vi "Param_Cmds.vi"(4 "Timeout":u16, 5 "Target":u16, 8 "Release":u16, 9 "Vacuum":u16, 10 "Write":bool, 11 "Queue":refnum<queue>) -> ()   [LabVIEW 2026]
doc: "Use this template to build a VI to use as a subVI."
panel:
  # "ÕfÃ÷£º°´ Write r°ÑËÄ¢µÏÞÖÆ¹ úáá·ÅßMÐÁÐ¡£"
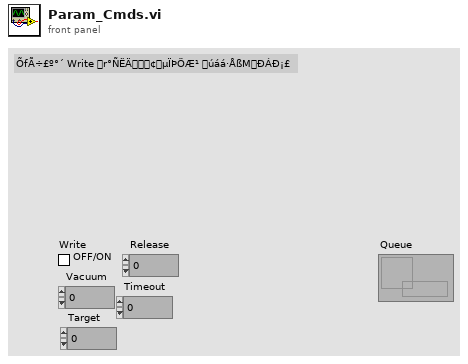
[diagram p1: front panel]
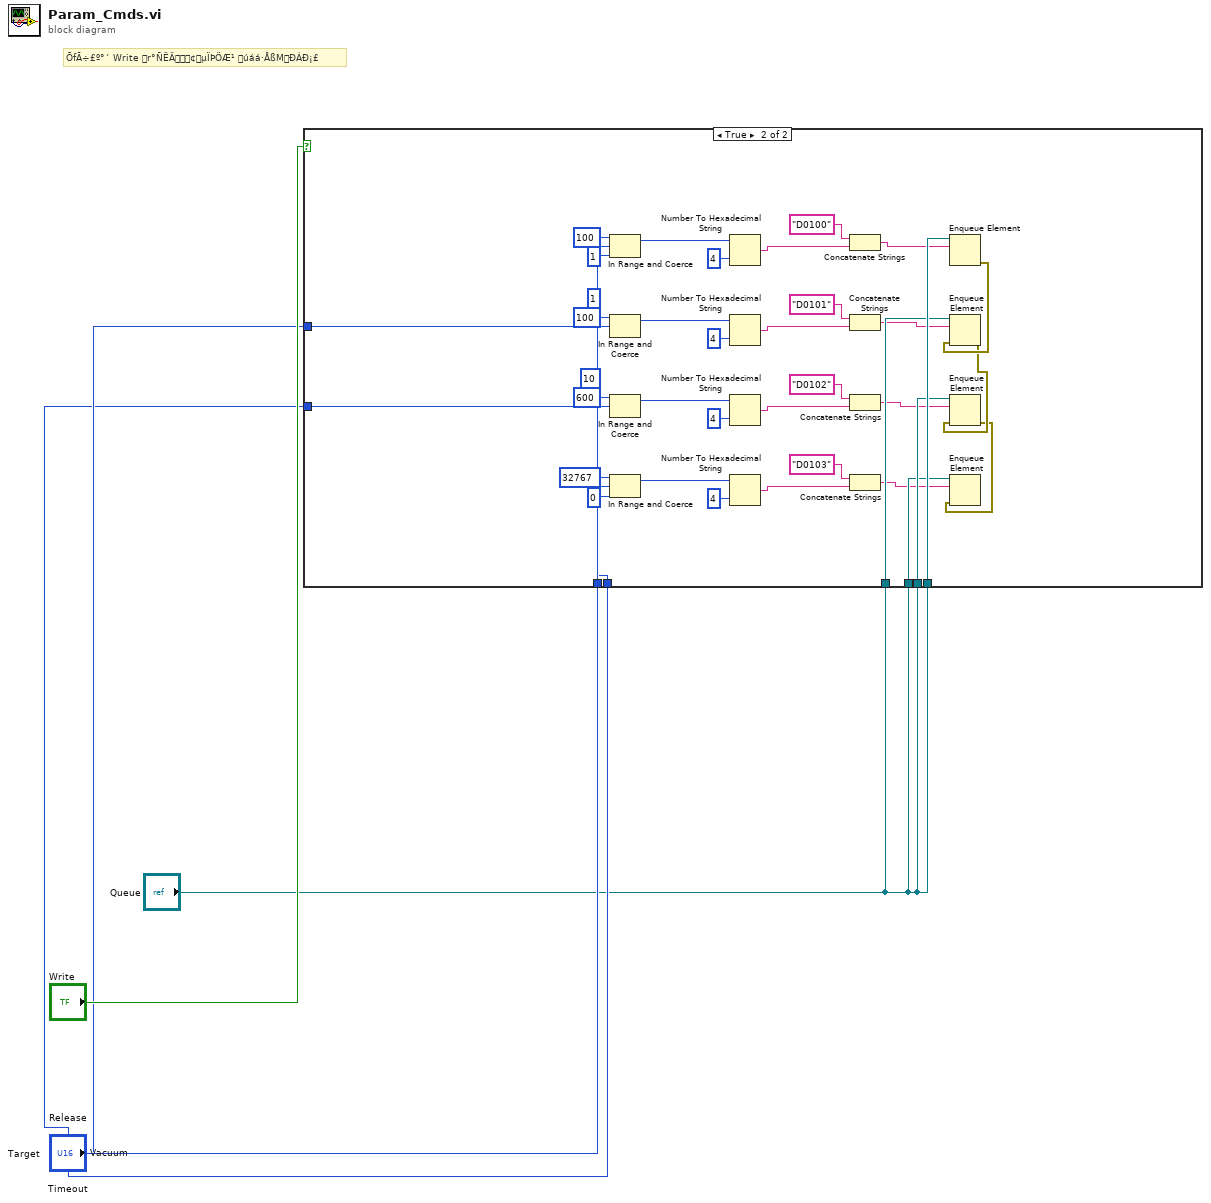
[diagram p0: block diagram]
diagram:
  # "ÕfÃ÷£º°´ Write r°ÑËÄ¢µÏÞÖÆ¹ úáá·ÅßMÐÁÐ¡£"
  n1 = case shown="True" "Write" {
    tunnel: "Vacuum" -> [_ w45]
    tunnel: "Queue" -> [_ w38]
    tunnel: "Release" -> [_ w36]
    tunnel: "Queue" -> [_ w29]
    tunnel: "Timeout" -> [_ w26]
    tunnel: "Queue" -> [_ w19]
    tunnel: "Target" -> [_ w16]
    tunnel: "Queue" -> [_ w9]
    frame False {
    }
    frame True {
      n2 = In Range and Coerce(upper limit=u16 100, x=w45, lower limit=u16 1) -> (coerced(x)=w42:u16)  [unwired: 1 out]
      n3 = In Range and Coerce(upper limit=u16 100, x=w36, lower limit=u16 1) -> (coerced(x)=w33:u16)  [unwired: 1 out]
      n4 = In Range and Coerce(upper limit=u16 600, x=w26, lower limit=u16 10) -> (coerced(x)=w23:u16)  [unwired: 1 out]
      n5 = In Range and Coerce(upper limit=u16 32767, x=w16, lower limit=u16 0) -> (coerced(x)=w13:u16)  [unwired: 1 out]
      n6 = Number To Hexadecimal String(1:i16 4 ("width (-)"), 2:w42) -> (0:w39:string)
      n7 = Number To Hexadecimal String(1:i16 4 ("width (-)"), 2:w33) -> (0:w30:string)
      n8 = Number To Hexadecimal String(1:i16 4 ("width (-)"), 2:w23) -> (0:w20:string)
      n9 = Number To Hexadecimal String(1:i16 4 ("width (-)"), 2:w13) -> (0:w10:string)
      n10 = Concatenate Strings("D0100", w39) -> (w37:string)
      n11 = Concatenate Strings("D0101", w30) -> (w28:string)
      n12 = Concatenate Strings("D0102", w20) -> (w18:string)
      n13 = Concatenate Strings("D0103", w10) -> (w8:string)
      n14 = Enqueue Element(queue=w38, element=w37) -> (error out=w27:errorcluster)  [unwired: 2 in, 2 out]
      n15 = Enqueue Element(queue=w29, element=w28, error in (no error)=w27) -> (error out=w17:errorcluster)  [unwired: 1 in, 2 out]
      n16 = Enqueue Element(queue=w19, element=w18, error in (no error)=w17) -> (error out=w7:errorcluster)  [unwired: 1 in, 2 out]
      n17 = Enqueue Element(queue=w9, element=w8, error in (no error)=w7) -> ()  [unwired: 1 in, 3 out]
    }
  }
